vi "Day 6.vi"() -> ()   [LabVIEW 2021]
uses:
  <vilib>/Utility/file.llb/Read Delimited Spreadsheet (I64).vi
panel:
  out "Results (Part 2)":map{i32, i64}(c390)
  out "Solution":i64
  out "Input":i32[](array[numeric])
  in  "Input File":enum32{"example input", "input"}(radio)
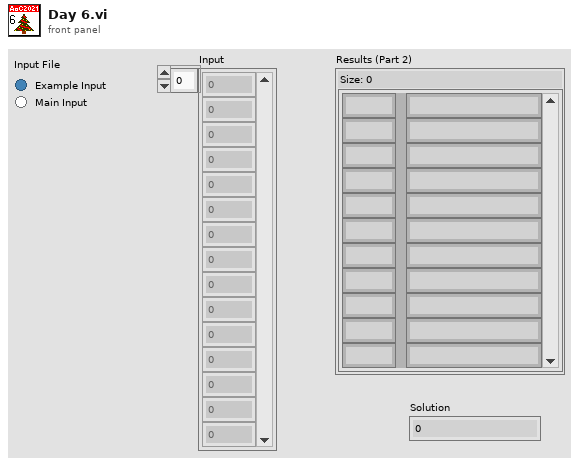
[diagram p1: front panel]
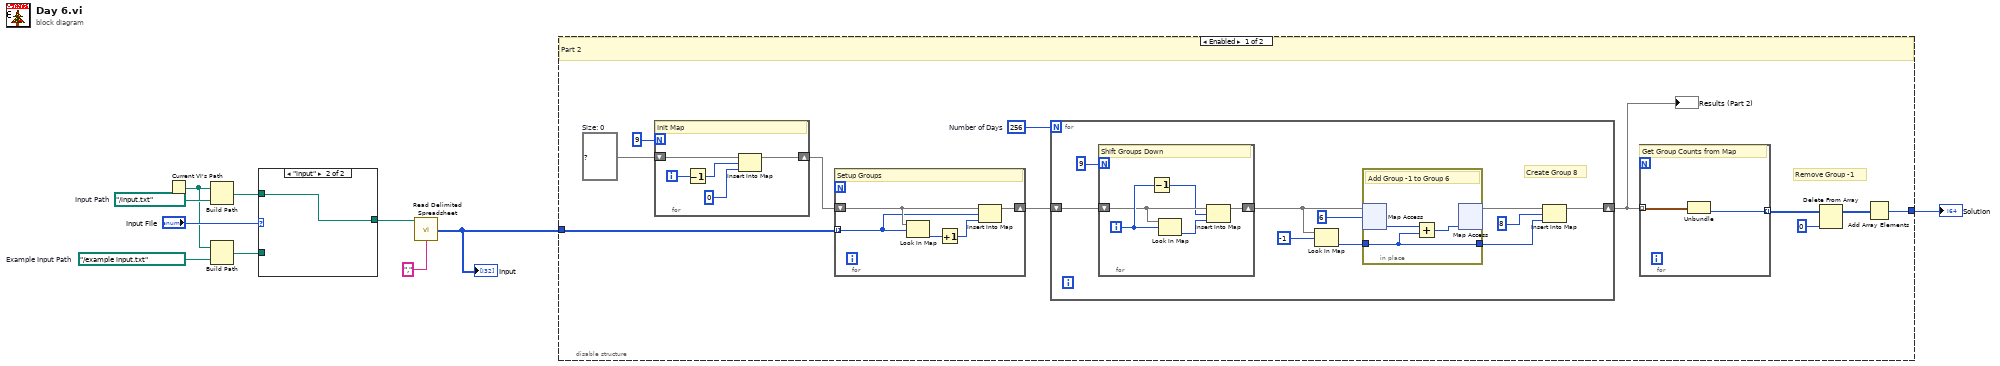
[diagram p0: block diagram]
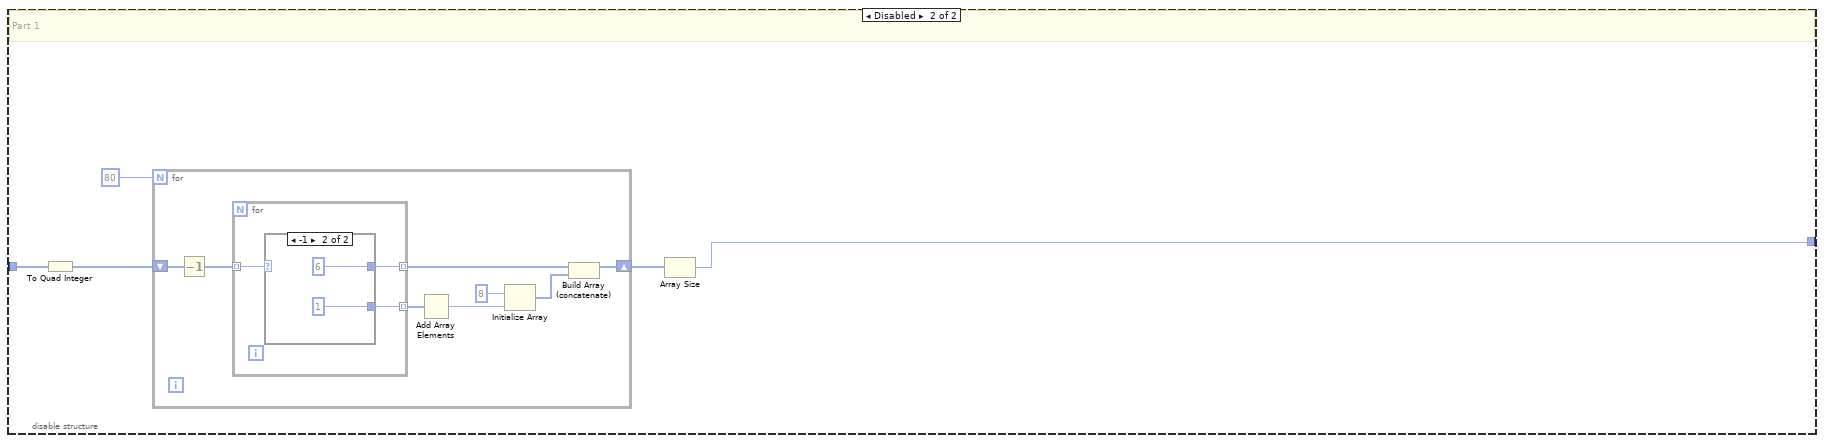
[diagram p3: hidden frame]
diagram:
  w9 = path "../example input.txt"  # Example Input Path
  w10 = path "../input.txt"  # Input Path
  n1 = Current VI's Path() -> (path=w4:path)
  n2 = Build Path(base path=w4, name or relative path=w10) -> (appended path=w7:path)
  n3 = Build Path(base path=w4, name or relative path=w9) -> (appended path=w6:path)
  n4 = case shown="\"input\"" "Input File" {
    tunnel: w7 -> [_ w12]
    tunnel: w6 -> [w11 _]
    tunnel: [w11 w12] -> w5
    frame "example input" {
    }
    frame "input" {
    }
  }
  n5 = call-poly <vilib>:"Read Delimited Spreadsheet.vi"("file path (dialog if empty)"=w5, "delimiter (\\t)"="," ("delimiter (\\t)")) -> ("first row"=w3:i64[])  [unwired: 8 in, 5 out]
  "Input" <- w3
  n6 = disable-structure shown="Enabled" {
    disable-tunnel: w3 -> [w22 w58]
    disable-tunnel: [w18 w55] -> w1
    frame Enabled {
      w14 = map{i32, i64} {}  # Size: 0
      w23 = 256  # Number of Days
      # "Remove Group -1"
      # "Part 2"
      n7 = for {
        N: 9 -> [_]
        shift-right: [w24] -> w13
        shift-left: w14 -> [w27]
        i -> [w28]
        # "Init Map"
        n8 = Decrement(x=w28) -> (x-1=w26:i32)
        n9 = Insert Into Map(map in=w27, key=w26, value=0) -> (map out=w24:map{i32, i64})  [unwired: 2 out]
      }
      n10 = for {
        tunnel: w22 -> [w29] mode=indexing
        shift-right: [w32] -> w21
        shift-left: w13 -> [w33]
        # "Setup Groups"
        n11 = Look In Map(map=w33, key=w29) -> (value=w31:i64)  [unwired: 1 in, 1 out]
        n12 = Increment(x=w31) -> (x+1=w30:i64)
        n13 = Insert Into Map(map in=w33, key=w29, value=w30) -> (map out=w32:map{i32, i64})  [unwired: 2 out]
      }
      n14 = for {
        N: w23 -> [_]
        shift-right: [w34] -> w20
        shift-left: w21 -> [w43]
        # "Create Group 8"
        n15 = for {
          N: 9 -> [_]
          shift-right: [w47] -> w41
          shift-left: w43 -> [w49]
          i -> [w51]
          # "Shift Groups Down"
          n16 = Decrement(x=w51) -> (x-1=w48:i32)
          n17 = Look In Map(map=w49, key=w51) -> (value=w50:i64)  [unwired: 1 in, 1 out]
          n18 = Insert Into Map(map in=w49, key=w48, value=w50) -> (map out=w47:map{i32, i64})  [unwired: 2 out]
        }
        n19 = Look In Map(map=w41, key=-1) -> (value=w39:i64)  [unwired: 1 in, 1 out]
        n20 = in-place {
          in-place-border: w39 -> [w45]
          in-place-border: [w45] -> w36
          # "Add Group -1 to Group 6"
          n21 = in-place-map #1(w41, 6) -> (w46:i64)  [unwired: 1 in, 1 out]
          n22 = Add(x=w46, y=w45) -> (x+y=w44:i64)
          n23 = in-place-map #1(w44) -> (w37:map{i32, i64})  [unwired: 1 in, 2 out]
        }
        n24 = Insert Into Map(map in=w37, key=8, value=w36) -> (map out=w34:map{i32, i64})  [unwired: 2 out]
      }
      "Results (Part 2)" <- w20
      n25 = for {
        tunnel: w20 -> [w53] mode=indexing
        tunnel: [w52] -> w19 mode=indexing
        # "Get Group Counts from Map"
        n26 = Unbundle(w53) -> (w52:i64)  [unwired: 1 out]
      }
      n27 = Delete From Array(array=w19, index=0) -> (array with subset deleted=w17:i64[])  [unwired: 1 in, 1 out]
      n28 = Add Array Elements(numeric array=w17) -> (sum=w18:i64)
    }
    frame Disabled {
      # "Part 1"
      n29 = To Quad Integer(1:w58) -> (0:w54:i64[])
      n30 = for {
        N: 80 -> [_]
        shift-right: [w60] -> w56
        shift-left: w54 -> [w66]
        n31 = Decrement(x=w66) -> (x-1=w65:i64[])
        n32 = for {
          tunnel: w65 -> [w69] mode=indexing
          tunnel: [w68] -> w64 mode=indexing
          tunnel: [w67] -> w63 mode=indexing
          n33 = case shown="-1" w69 {
            selector: w69 -> [w70 _]
            tunnel: [w70 6] -> w68
            tunnel: [_ 1] -> w67
            frame Default {
            }
            frame -1 {
            }
          }
        }
        n34 = Add Array Elements(numeric array=w63) -> (sum=w62:i32)
        n35 = Initialize Array(8, w62) -> (w59:i32[])
        n36 = Build Array (concatenate)(w64, w59) -> (w60:i64[])
      }
      n37 = Array Size(array=w56) -> (size(s)=w55:i32)
    }
  }
  "Solution" <- w1
